vi "Close.vi"(8 "error in (no error)":errorcluster, 11 "ActivationHandler in":refnum<class "ActivationHandler.lvclass">) -> (0 "error out":errorcluster)   [LabVIEW 2026, in "ToastNotification.lvlib" / "ActivationHandler.lvclass"]
doc: "Cleanup hook for activation handlers. The base implementation does not own resources. Override in a child class to release resources acquired by Initialize. ToastService.Close invokes this hook. Implement cleanup so incoming errors do not prevent release; define how callback activity is stopped before resources are destroyed."
uses:
  ActivationHandler.lvclass
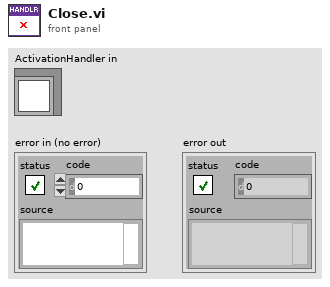
[diagram p1: front panel]
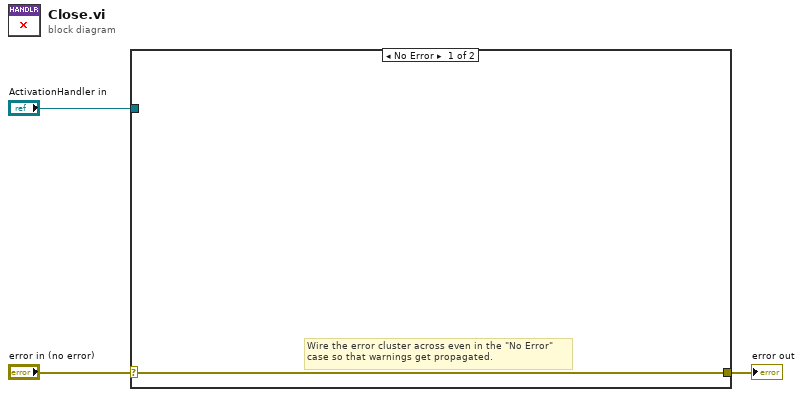
[diagram p0: block diagram]
diagram:
  n1 = case shown="No Error" "error in (no error)" {
    selector: "error in (no error)" -> [w4 w5]
    tunnel: [w4 w5] -> w2
    tunnel: "ActivationHandler in" -> [_ _]
    frame No Error {
      # "Wire the error cluster across even in the \"No Error\"\ncase so that warnings get propagated."
    }
    frame Error {
    }
  }
  "error out" <- w2
